vi "1f.fibre_optic_Distriubuted_strain_sensing_system.vi"() -> ()   [LabVIEW 2017]
uses:
  <vilib>/Instr/_visa.llb/VISA Configure Serial Port (Instr).vi
panel:
  out "Strain Resolution":string
  out "hZ":dbl
  out "?":cluster{dbl[], u16[]}(graph)
  # "REAL TIME FIBER OPTIC STRUCTURAL HEALTH MONITORING SYSTEM"
  # "COPY RIGHT : Dr Vishnu Prasad"
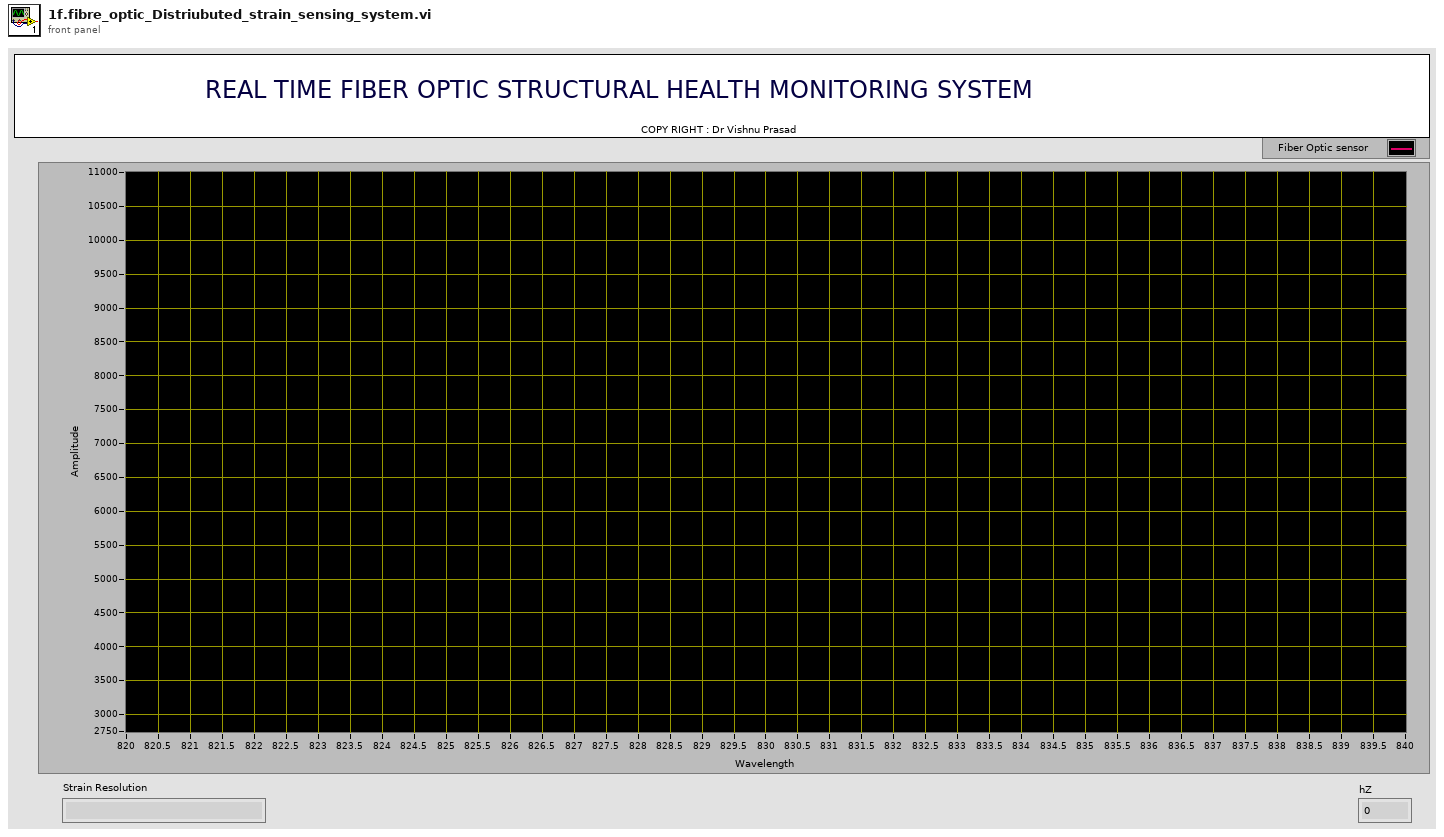
[diagram p1: front panel]
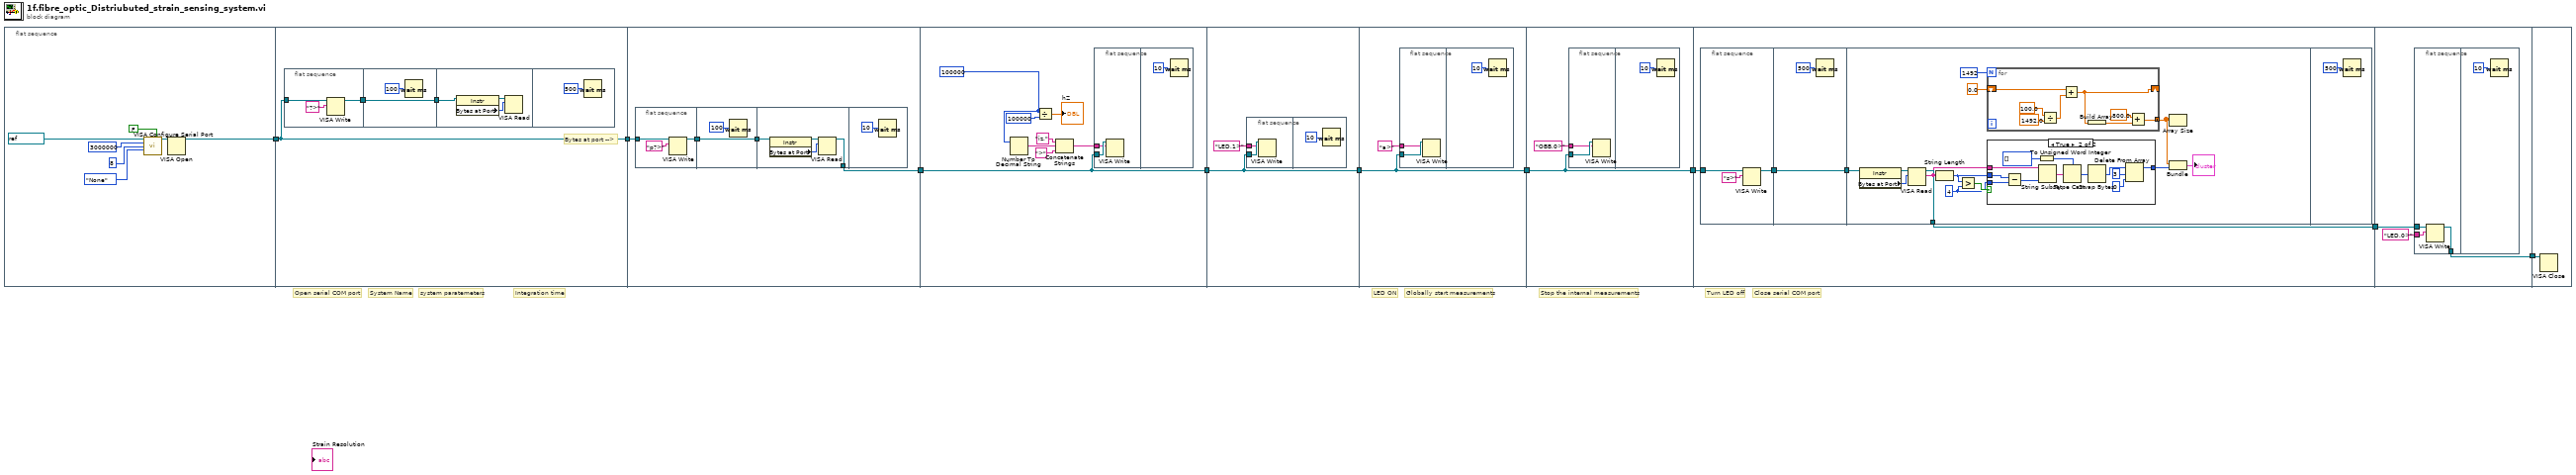
[diagram p0: block diagram]
diagram:
  # "Globally start measurements"
  # "LED ON"
  # "System Name"
  # "Integration time"
  # "system paratemeters"
  # "Close serial COM port"
  # "Turn LED off"
  # "Stop the internal measurements"
  # "Open serial COM port"
  n1 = flat-sequence {
    tunnel: [w11] -> w1
    tunnel: [w17] -> w9
    tunnel: w1 -> [w17]
    tunnel: w9 -> [w30]
    tunnel: [w29] -> w8
    tunnel: w8 -> [w46]
    tunnel: [w46] -> w7
    tunnel: w7 -> [w54]
    tunnel: [w54] -> w2
    tunnel: [w59] -> w6
    tunnel: w2 -> [w59]
    tunnel: w6 -> [w64]
    tunnel: [w64] -> w5
    tunnel: w5 -> [w70]
    tunnel: [w69] -> w4
    tunnel: w4 -> [w113]
    tunnel: [w112] -> w3
    tunnel: w3 -> [w119]
    frame #0 {
      n2 = call-poly "VISA Configure Serial Port"("VISA resource name"=refnum<visa-resource-name> "COM7", "Enable Termination\nChar (T)"=FALSE ("Enable Termination\nChar (T)"), "baud rate (9600)"=u32 3000000, "data bits (8)"=u16 8, "parity (0:none)"=enum16{"None", "Odd", "Even", "Mark", "Space"}."None") -> ("VISA resource name out"=w16:refnum<visa-resource-name>)  [unwired: 9 in, 1 out]
      n3 = VISA Open(VISA resource name=w16) -> (VISA resource name=w11:refnum<visa-resource-name>)  [unwired: 4 in, 1 out]
    }
    frame #1 {
      # "Bytes at port -->"
      n4 = flat-sequence {
        tunnel: [w22] -> w19
        tunnel: w17 -> [w21]
        tunnel: [w23] -> w18
        tunnel: w19 -> [w23]
        tunnel: w18 -> [w27]
        frame #0 {
          n5 = VISA Write(VISA resource name=w21, write buffer="?>") -> (VISA resource name out=w22:refnum<visa-resource-name>)  [unwired: 1 in, 2 out]
        }
        frame #1 {
          n6 = Wait (ms)(milliseconds to wait=u32 100 ("Zu wartende ms")) -> ()  [unwired: 1 out]
        }
        frame #2 {
          n7 = property class="Instr"(reference=w27) -> (reference out=w26:refnum<visa-resource-name>, "Bytes at Port"=w25:u32)  [unwired: 1 in, 1 out]
          n8 = VISA Read(VISA resource name=w26, byte count=w25) -> ()  [unwired: 1 in, 4 out]
        }
        frame #3 {
          n9 = Wait (ms)(milliseconds to wait=u32 500 ("Zu wartende ms")) -> ()  [unwired: 1 out]
        }
      }
    }
    frame #2 {
      n10 = flat-sequence {
        tunnel: [w35] -> w32
        tunnel: w30 -> [w33]
        tunnel: [w36] -> w31
        tunnel: w32 -> [w36]
        tunnel: w31 -> [w41]
        tunnel: [w38] -> w29
        frame #0 {
          n11 = VISA Write(VISA resource name=w33, write buffer="p?>") -> (VISA resource name out=w35:refnum<visa-resource-name>)  [unwired: 1 in, 2 out]
        }
        frame #1 {
          n12 = Wait (ms)(milliseconds to wait=u32 100 ("Zu wartende ms")) -> ()  [unwired: 1 out]
        }
        frame #2 {
          n13 = property class="Instr"(reference=w41) -> (reference out=w40:refnum<visa-resource-name>, "Bytes at Port"=w39:u32)  [unwired: 1 in, 1 out]
          n14 = VISA Read(VISA resource name=w40, byte count=w39) -> (VISA resource name out=w38:refnum<visa-resource-name>)  [unwired: 1 in, 3 out]
        }
        frame #3 {
          n15 = Wait (ms)(milliseconds to wait=u32 10 ("Zu wartende ms")) -> ()  [unwired: 1 out]
        }
      }
    }
    frame #3 {
      w43 = 100000 ("Integration time (µs) 2")
      n16 = Number To Decimal String(number=w43) -> (decimal integer string=w50:string)  [unwired: 1 in]
      n17 = Divide(x=w43, y=100000) -> (x/y=→"hZ":dbl)
      n18 = Concatenate Strings("iz," ("String"), w50, ">" ("String")) -> (w47:string)
      n19 = flat-sequence {
        tunnel: w46 -> [w52]
        tunnel: w47 -> [w51]
        frame #0 {
          n20 = VISA Write(VISA resource name=w52, write buffer=w51) -> ()  [unwired: 1 in, 3 out]
        }
        frame #1 {
          n21 = Wait (ms)(milliseconds to wait=u32 10 ("Zu wartende ms")) -> ()  [unwired: 1 out]
        }
      }
    }
    frame #4 {
      n22 = flat-sequence {
        tunnel: w54 -> [w57]
        tunnel: "LED,1>" ("String") -> [w56]
        frame #0 {
          n23 = VISA Write(VISA resource name=w57, write buffer=w56) -> ()  [unwired: 1 in, 3 out]
        }
        frame #1 {
          n24 = Wait (ms)(milliseconds to wait=u32 10 ("Zu wartende ms")) -> ()  [unwired: 1 out]
        }
      }
    }
    frame #5 {
      n25 = flat-sequence {
        tunnel: w59 -> [w62]
        tunnel: "a>" ("String") -> [w61]
        frame #0 {
          n26 = VISA Write(VISA resource name=w62, write buffer=w61) -> ()  [unwired: 1 in, 3 out]
        }
        frame #1 {
          n27 = Wait (ms)(milliseconds to wait=u32 10 ("Zu wartende ms")) -> ()  [unwired: 1 out]
        }
      }
    }
    frame #6 {
      n28 = flat-sequence {
        tunnel: w64 -> [w67]
        tunnel: "OBB,0>" ("String") -> [w66]
        frame #0 {
          n29 = VISA Write(VISA resource name=w67, write buffer=w66) -> ()  [unwired: 1 in, 3 out]
        }
        frame #1 {
          n30 = Wait (ms)(milliseconds to wait=u32 10 ("Zu wartende ms")) -> ()  [unwired: 1 out]
        }
      }
    }
    frame #7 {
      n31 = flat-sequence {
        tunnel: [w75] -> w72
        tunnel: w70 -> [w73]
        tunnel: [w76] -> w71
        tunnel: w72 -> [w76]
        tunnel: w71 -> [w85]
        tunnel: [w84] -> w69
        frame #0 {
          n32 = VISA Write(VISA resource name=w73, write buffer="s>") -> (VISA resource name out=w75:refnum<visa-resource-name>)  [unwired: 1 in, 2 out]
        }
        frame #1 {
          n33 = Wait (ms)(milliseconds to wait=u32 500 ("Zu wartende ms")) -> ()  [unwired: 1 out]
        }
        frame #2 {
          w78 = 4 ("y")
          n34 = property class="Instr"(reference=w85) -> (reference out=w83:refnum<visa-resource-name>, "Bytes at Port"=w82:u32)  [unwired: 1 in, 1 out]
          n35 = VISA Read(VISA resource name=w83, byte count=w82) -> (VISA resource name out=w84:refnum<visa-resource-name>, read buffer=w81:string)  [unwired: 1 in, 2 out]
          n36 = String Length(string=w81) -> (length=w80:i32)
          n37 = Greater?(x=w80, y=w78) -> (0:w79:bool)
          n38 = for {
            N: 1492 -> [_]
            shift-right: [w109] -> _
            shift-left: 0.0 -> [w110]
            tunnel: [w106] -> w90 mode=concatenating
            n39 = Divide(x=100.0 ("x/y"), y=1492.0) -> (x/y=w103:dbl)
            n40 = Add(x=w110, y=w103) -> (x+y=w109:dbl)
            n41 = Build Array(w109) -> (w107:dbl[])
            n42 = Add(x=800.0 ("x+y"), y=w107) -> (x+y=w106:dbl[])
          }
          n43 = case shown="True" w79 {
            tunnel: w81 -> [_ w102]
            tunnel: w80 -> [_ w101]
            tunnel: w78 -> [_ w100]
            tunnel: [_ w91] -> w88
            frame False {
            }
            frame True {
              n44 = Subtract(x=w101, y=w100) -> (x-y=w99:i32)
              n45 = To Unsigned Word Integer(number=i32[] []) -> (unsigned 16bit integer=w98:u16[])
              n46 = String Subset(string=w102, length (rest)=w99) -> (substring=w97:string)  [unwired: 1 in]
              n47 = Type Cast(type=w98, x=w97) -> (*(type *) &x=w95:u16[])
              n48 = Swap Bytes(anything=w95) -> (byte swapped=w94:u16[])
              n49 = Delete From Array(array=w94, length=3, index=0) -> (array with subset deleted=w91:u16[])  [unwired: 1 out]
            }
          }
          n50 = Array Size(array=w90) -> ()  [unwired: 1 out]
          n51 = Bundle(w90, w88) -> (→"?":cluster{dbl[], u16[]})  [unwired: 1 in]
        }
        frame #3 {
          n52 = Wait (ms)(milliseconds to wait=u32 500 ("Zu wartende ms")) -> ()  [unwired: 1 out]
        }
      }
    }
    frame #8 {
      n53 = flat-sequence {
        tunnel: w113 -> [w117]
        tunnel: "LED,0>" ("String") -> [w116]
        tunnel: [w115] -> w112
        frame #0 {
          n54 = VISA Write(VISA resource name=w117, write buffer=w116) -> (VISA resource name out=w115:refnum<visa-resource-name>)  [unwired: 1 in, 2 out]
        }
        frame #1 {
          n55 = Wait (ms)(milliseconds to wait=u32 10 ("Zu wartende ms")) -> ()  [unwired: 1 out]
        }
      }
    }
    frame #9 {
      n56 = VISA Close(VISA resource name=w119) -> ()  [unwired: 1 in, 1 out]
    }
  }
